vi "Prepend Text to Item Name.vi"(11 "Item Name":string) -> (3 "Item Name out":string)   [LabVIEW 2020, in "VI Properties Editor.lvlib"]
doc: "Prepends text to <B>Item Name</B> to show that it has been modified."
uses:
  VI Properties Editor.lvlib
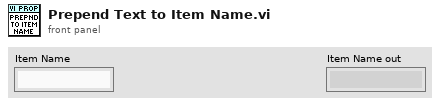
[diagram p1: front panel]
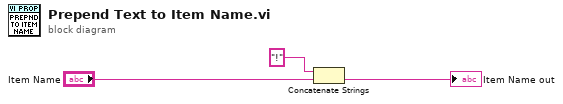
[diagram p0: block diagram]
diagram:
  n1 = Concatenate Strings("!" ("format string"), "Item Name") -> (→"Item Name out":string)
